vi "RemoteVI Complex Fixture Events.vi"(0 "Panel":refnum<vi>, 11 "error in":errorcluster) -> (15 "error out":errorcluster)   [LabVIEW 2020]
doc: "Event loop of RemoteVI Complex Fixture.vi, a subVI so that the fixture's own diagram has no Event Structure (its panel is grafted from another VI, and only static Value Change events survive that). Finds the controls by label on Panel (RemoteVI Complex Fixture Find Controls.vi, every pane, tab page and cluster), registers Value Change, Mouse Down and Mouse Up of each and sends one log line per event through the named queue RemoteVI Complex Fixture: value lines (RemoteVI Complex Fixture Value Text.vi: every Val of the value's XML joined with |), mousedown and mouseup lines. Stop sends the named notifier RemoteVI Complex Fixture and ends the loop. Inspector opens RemoteVI Complex Inspector.vi in its own window (FP.Open without activating, Run VI). View shows View A or View B in the subpanel Viewer. Stop and Inspector are switches set back to FALSE here, because a latched button only resets when its terminal is read."
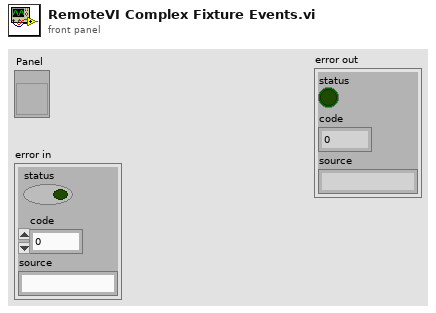
[diagram p1: front panel]
types:
  T1 = typedef "LVPoint32TypeDef.ctl" = cluster{"Horizontal":i32, "Vertical":i32}
  T2 = cluster{"Shift":bool, "Ctrl":bool, "Alt":bool, "Cmd":bool, "Opt":bool}
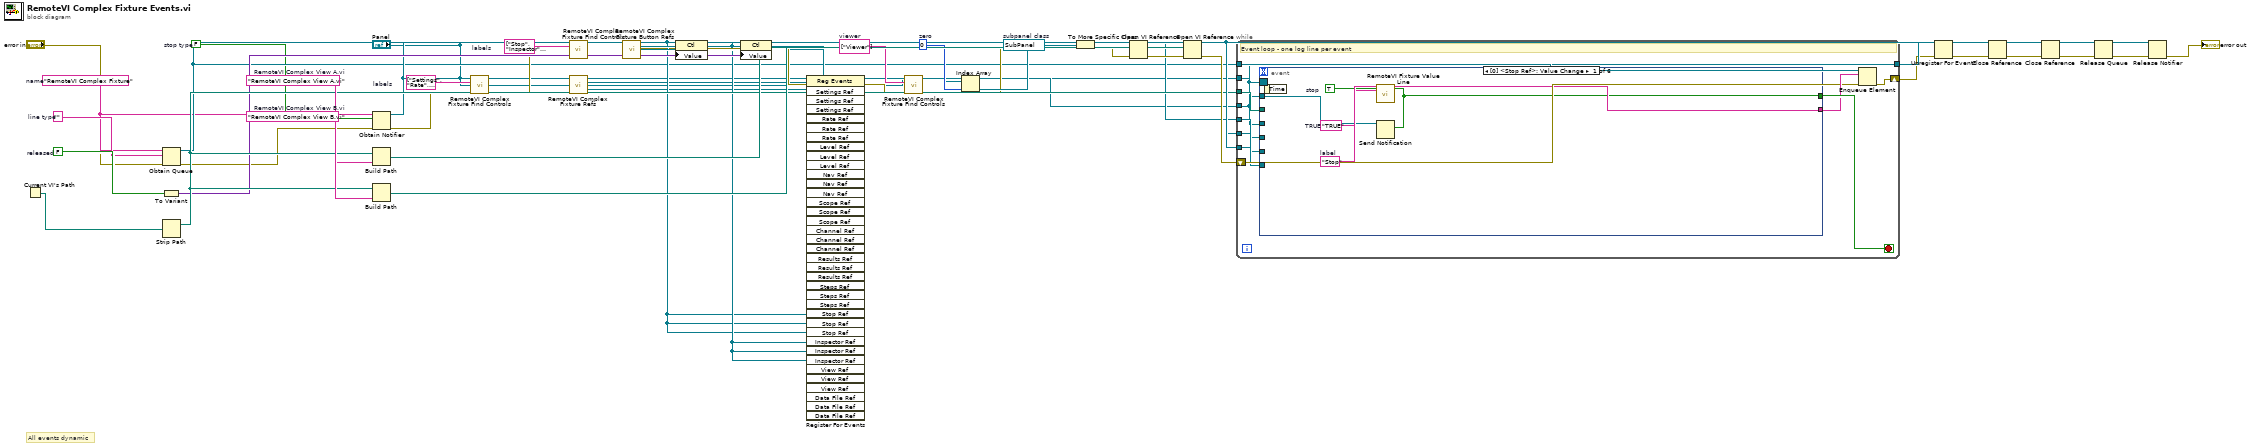
[diagram p0: block diagram]
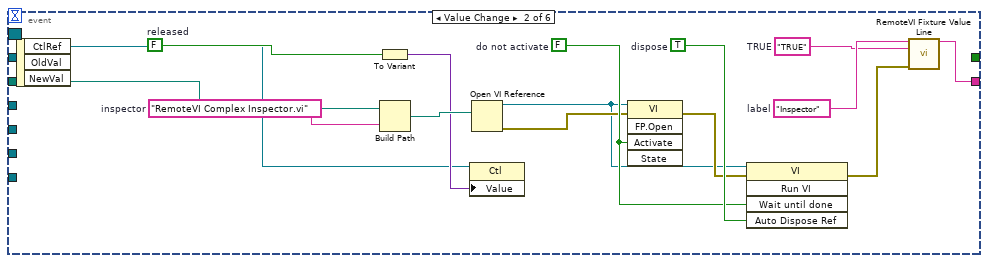
[diagram p2: hidden frame]
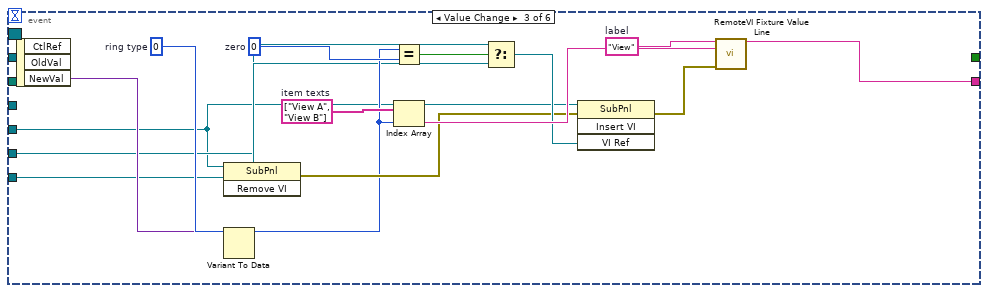
[diagram p3: hidden frame]
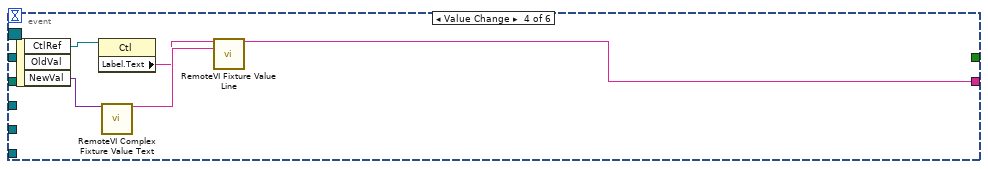
[diagram p4: hidden frame]
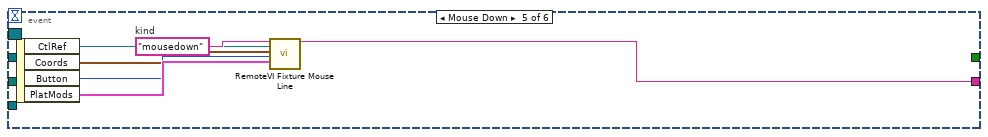
[diagram p5: hidden frame]
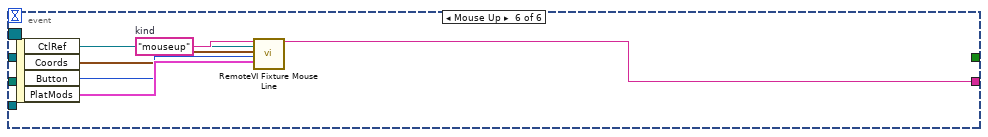
[diagram p6: hidden frame]
diagram:
  w46 = "RemoteVI Complex View B.vi"  # RemoteVI Complex View B.vi
  w44 = "RemoteVI Complex View A.vi"  # RemoteVI Complex View A.vi
  w39 = refnum<vi> refnum  # subpanel class
  w37 = 0  # zero
  w34 = string[] ["Viewer"]  # viewer
  w28 = FALSE  # released
  w13 = string[] ["Stop", "Inspector", "View", "Data File"]  # labels
  w10 = string[] ["Settings", "Rate", "Level", "Nav", "Scope", "Channel", "Results", "Steps"]  # labels
  w5 = FALSE  # stop type
  w4 = ""  # line type
  w3 = "RemoteVI Complex Fixture"  # name
  # "All events dynamic"
  n1 = Current VI's Path() -> (path=w42:path)
  n2 = Obtain Queue(name (unnamed)=w3, element data type=w4, error in (no error)="error in") -> (queue out=w6:refnum<queue>, error out=w7:errorcluster)  [unwired: 2 in, 1 out]
  n3 = To Variant(anything=w28) -> (Variant=w29:variant)
  n4 = Strip Path(path=w42) -> (stripped path=w43:path)  [unwired: 1 out]
  n5 = Obtain Notifier(name (unnamed)=w3, notification data type=w5, error in (no error)=w7) -> (notifier out=w8:refnum<notifier>, error out=w9:errorcluster)  [unwired: 1 in, 1 out]
  n6 = Build Path(base path=w43, name or relative path=w44) -> (appended path=w45:path)
  n7 = Build Path(base path=w43, name or relative path=w46) -> (appended path=w47:path)
  n8 = call "RemoteVI Complex Fixture Find Controls.vi"("Panel"="Panel", "labels"=w10, "error in"=w9) -> ("Controls"=w11:refnum<vi>[], "error out"=w12:errorcluster)  [unwired: 11 in]
  n9 = call "RemoteVI Complex Fixture Find Controls.vi"("Panel"="Panel", "labels"=w13, "error in"=w12) -> ("Controls"=w14:refnum<vi>[], "error out"=w15:errorcluster)  [unwired: 11 in]
  n10 = call "RemoteVI Complex Fixture Refs.vi"("Controls"=w11) -> ("Settings Ref"=w16:refnum<vi>, "Rate Ref"=w17:refnum<vi>, "Level Ref"=w18:refnum<vi>, "Nav Ref"=w19:refnum<vi>, "Scope Ref"=w20:refnum<vi>, "Channel Ref"=w21:refnum<vi>, "Results Ref"=w22:refnum<vi>, "Steps Ref"=w23:refnum<vi>)  [unwired: 7 in]
  n11 = call "RemoteVI Complex Fixture Button Refs.vi"("Controls"=w14) -> ("Stop Ref"=w24:refnum<vi>, "Inspector Ref"=w25:refnum<vi>, "View Ref"=w26:refnum<vi>, "Data File Ref"=w27:refnum<vi>)  [unwired: 11 in]
  n12 = property class="Ctl"(reference=w24, error in=w15, "Value"=w29) -> (error out=w30:errorcluster)  [unwired: 1 out]
  n13 = property class="Ctl"(reference=w25, error in=w30, "Value"=w29) -> (error out=w31:errorcluster)  [unwired: 1 out]
  n14 = register-events(error in=w31, w16, w16, w16, w17, w17, w17, w18, w18, w18, w19, w19, w19, w20, w20, w20, w21, w21, w21, w22, w22, w22, w23, w23, w23, w24, w24, w24, w25, w25, w25, w26, w26, w26, w27, w27, w27) -> (reference out=w32:refnum<event-registration>, error out=w33:errorcluster)  [unwired: 1 in]
  n15 = call "RemoteVI Complex Fixture Find Controls.vi"("Panel"="Panel", "labels"=w34, "error in"=w33) -> ("Controls"=w35:refnum<vi>[], "error out"=w36:errorcluster)  [unwired: 11 in]
  n16 = Index Array(array=w35, index=w37) -> (element=w38:refnum<vi>)
  n17 = To More Specific Class(target class=w39, reference=w38, error in=w36) -> (specific class reference=w40:refnum<vi>, error out=w41:errorcluster)
  n18 = Open VI Reference(vi path=w45, error in (no error)=w41) -> (vi reference=w48:refnum<vi>, error out=w49:errorcluster)  [unwired: 4 in]
  n19 = Open VI Reference(vi path=w47, error in (no error)=w49) -> (vi reference=w50:refnum<vi>, error out=w51:errorcluster)  [unwired: 4 in]
  n20 = while {
    tunnel: w6 -> [w65]
    tunnel: w8 -> [w59]
    tunnel: w43 -> [w64]
    tunnel: w32 -> [w60]
    tunnel: [w60] -> w53
    tunnel: w40 -> [w61]
    tunnel: w48 -> [w62]
    tunnel: w50 -> [w63]
    shift-right: [w67] -> w52
    shift-left: w51 -> [w66]
    stop <- w69 stop-if-true
    # "Event loop - one log line per event"
    n21 = event shown="[0] <Stop Ref>: Value Change" {
      selector: w60 -> [_ _ _ _ _ _]
      dyn-events: _ -> [_ _ _ _ _ _]
      timeout: _ -> [_ _ _ _ _ _]
      tunnel: [w71 _ _ _ _ _] -> w69
      tunnel: [w74 w89 w104 w109 w115 w121] -> w68
      tunnel: w59 -> [w70 _ _ _ _ _]
      tunnel: w64 -> [_ w75 _ _ _ _]
      tunnel: w60 -> [_ _ _ _ _ _]
      tunnel: w61 -> [_ _ w90 _ _ _]
      tunnel: w62 -> [_ _ w91 _ _ _]
      tunnel: w63 -> [_ _ w92 _ _ _]
      event Value Change {
        w73 = "Stop"  # label
        w72 = "TRUE"  # TRUE
        w71 = TRUE  # stop
        n22 = event-data() -> ()  [unwired: 1 in, 1 out]
        n23 = call "RemoteVI Fixture Value Line.vi"("label"=w73, "value"=w72) -> ("line"=w74:string)  [unwired: 12 in, 1 out]
        n24 = Send Notification(notification=w71, notifier=w70) -> ()  [unwired: 1 in, 2 out]
      }
      event Value Change {
        w88 = "Inspector"  # label
        w87 = "TRUE"  # TRUE
        w85 = TRUE  # dispose
        w83 = FALSE  # do not activate
        w79 = "RemoteVI Complex Inspector.vi"  # inspector
        w77 = FALSE  # released
        n25 = event-data() -> ("CtlRef"=w76:refnum<vi>)  [unwired: 1 in, 2 out]
        n26 = To Variant(anything=w77) -> (Variant=w78:variant)
        n27 = Build Path(base path=w75, name or relative path=w79) -> (appended path=w80:path)
        n28 = property class="Ctl"(reference=w76, "Value"=w78) -> ()  [unwired: 1 in, 2 out]
        n29 = Open VI Reference(vi path=w80) -> (vi reference=w81:refnum<vi>, error out=w82:errorcluster)  [unwired: 5 in]
        n30 = invoke class="VI" method="FP.Open"(reference=w81, error in=w82, "Activate"=w83) -> (error out=w84:errorcluster)  [unwired: 2 in, 4 out]
        n31 = invoke class="VI" method="Run VI"(reference=w81, error in=w84, "Wait until done"=w83, "Auto Dispose Ref"=w85) -> (error out=w86:errorcluster)  [unwired: 1 in, 4 out]
        n32 = call "RemoteVI Fixture Value Line.vi"("label"=w88, "value"=w87, "error in"=w86) -> ("line"=w89:string)  [unwired: 11 in, 1 out]
      }
      event Value Change {
        w103 = "View"  # label
        w101 = string[] ["View A", "View B"]  # item texts
        w97 = 0  # zero
        w94 = 0  # ring type
        n33 = event-data() -> ("NewVal"=w93:variant)  [unwired: 1 in, 2 out]
        n34 = invoke class="SubPnl" method="Remove VI"(reference=w90) -> (error out=w96:errorcluster)  [unwired: 2 in, 2 out]
        n35 = Variant To Data(type=w94, Variant=w93) -> (data=w95:i32)  [unwired: 1 in, 1 out]
        n36 = Equal?(x=w95, y=w97) -> (x = y?=w98:bool)
        n37 = Index Array(array=w101, index=w95) -> (element=w102:string)
        n38 = Select(t=w91, s=w98, f=w92) -> (s? t:f=w99:refnum<vi>)
        n39 = invoke class="SubPnl" method="Insert VI"(reference=w90, error in=w96, "VI Ref"=w99) -> (error out=w100:errorcluster)  [unwired: 1 in, 3 out]
        n40 = call "RemoteVI Fixture Value Line.vi"("label"=w103, "value"=w102, "error in"=w100) -> ("line"=w104:string)  [unwired: 11 in, 1 out]
      }
      event Value Change {
        n41 = event-data() -> ("CtlRef"=w105:refnum<vi>, "NewVal"=w106:variant)  [unwired: 1 in, 1 out]
        n42 = property class="Ctl"(reference=w105) -> ("Label.Text"=w107:string)  [unwired: 1 in, 2 out]
        n43 = call "RemoteVI Complex Fixture Value Text.vi"("value"=w106) -> ("text"=w108:string)  [unwired: 13 in, 1 out]
        n44 = call "RemoteVI Fixture Value Line.vi"("label"=w107, "value"=w108) -> ("line"=w109:string)  [unwired: 12 in, 1 out]
      }
      event Mouse Down {
        w114 = "mousedown"  # kind
        n45 = event-data() -> ("CtlRef"=w110:refnum<vi>, "Coords"=w111:T1, "Button"=w112:u16, "PlatMods"=w113:T2)  [unwired: 1 in]
        n46 = call "RemoteVI Fixture Mouse Line.vi"("kind"=w114, "CtlRef"=w110, "Coords"=w111, "Button"=w112, "PlatMods"=w113) -> ("line"=w115:string)  [unwired: 13 in, 1 out]
      }
      event Mouse Up {
        w120 = "mouseup"  # kind
        n47 = event-data() -> ("CtlRef"=w116:refnum<vi>, "Coords"=w117:T1, "Button"=w118:u16, "PlatMods"=w119:T2)  [unwired: 1 in]
        n48 = call "RemoteVI Fixture Mouse Line.vi"("kind"=w120, "CtlRef"=w116, "Coords"=w117, "Button"=w118, "PlatMods"=w119) -> ("line"=w121:string)  [unwired: 13 in, 1 out]
      }
    }
    n49 = Enqueue Element(queue=w65, element=w68, error in (no error)=w66) -> (error out=w67:errorcluster)  [unwired: 1 in, 2 out]
  }
  n50 = Unregister For Events(event registration refnum=w53, error in=w52) -> (error out=w54:errorcluster)
  n51 = Close Reference(reference=w48, error in (no error)=w54) -> (error out=w55:errorcluster)
  n52 = Close Reference(reference=w50, error in (no error)=w55) -> (error out=w56:errorcluster)
  n53 = Release Queue(queue=w6, error in (no error)=w56) -> (error out=w57:errorcluster)  [unwired: 1 in, 2 out]
  n54 = Release Notifier(notifier=w8, error in (no error)=w57) -> (error out=→"error out":errorcluster)  [unwired: 1 in, 2 out]
